vi "CIVI Query Once.vi"(10 "write buffer":string, 11 "VISA Refnum in":refnum<visa-resource-name>) -> (0 "error out":errorcluster, 3 "read buffer":string)   [LabVIEW 2026]
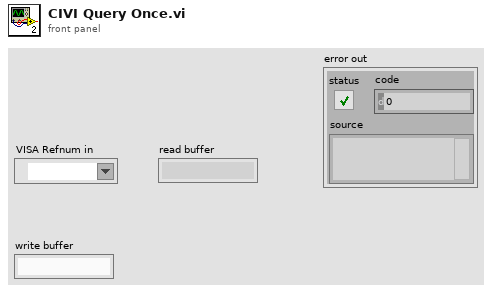
[diagram p1: front panel]
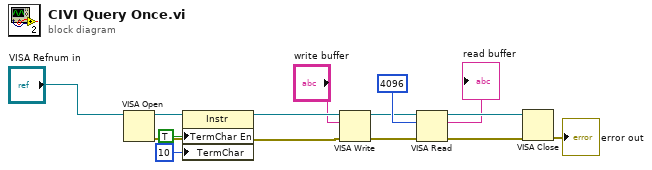
[diagram p0: block diagram]
diagram:
  n1 = VISA Open(VISA resource name="VISA Refnum in") -> (VISA resource name=w13:refnum<visa-resource-name>, error out=w10:errorcluster)  [unwired: 4 in]
  n2 = property class="Instr"(reference=w13, error in=w10, "TermChar En"=TRUE ("Message Based Settings:Termination Character Enable"), "TermChar"=u8 10 ("Message Based Settings:Termination Character")) -> (reference out=w12:refnum<visa-resource-name>, error out=w11:errorcluster)
  n3 = VISA Write(VISA resource name=w12, write buffer="write buffer", error in (no error)=w11) -> (VISA resource name out=w4:refnum<visa-resource-name>, error out=w6:errorcluster)  [unwired: 1 out]
  n4 = VISA Read(VISA resource name=w4, byte count=u32 4096, error in (no error)=w6) -> (VISA resource name out=w5:refnum<visa-resource-name>, read buffer=→"read buffer":string, error out=w7:errorcluster)  [unwired: 1 out]
  n5 = VISA Close(VISA resource name=w5, error in (no error)=w7) -> (error out=→"error out":errorcluster)
